vi "Convert API String Arguments to Data(variant).vi"(7 "Type":variant, 9 "error in (no error)":errorcluster, 10 "Strict Label Check?(T)":bool=TRUE, 11 "String":string) -> (1 "error":errorcluster, 3 "Data":variant)   [LabVIEW 2017, in "API String Arguments Support.lvlib"]
uses:
  API String Arguments Support.lvlib
  <vilib>/Utility/Data Type/Type Definitions/Data Type.ctl
  <vilib>/Utility/Data Type/Type Definitions/Tag Type.ctl
  <vilib>/Utility/Data Type/Type Definitions/Refnum Type.ctl
  <userlib>/_NEVSTOP/Communicable State Machine(CSM)/AdvanceAPI/CSM - Keywords.vi
  <vilib>/Utility/Data Type/NI_Data Type.lvlib
  <userlib>/_NEVSTOP/Communicable State Machine(CSM)/Communicable State Machine.lvlib
  <userlib>/_NEVSTOP/Communicable State Machine(CSM)/_Shared/CSM Shared.lvlib
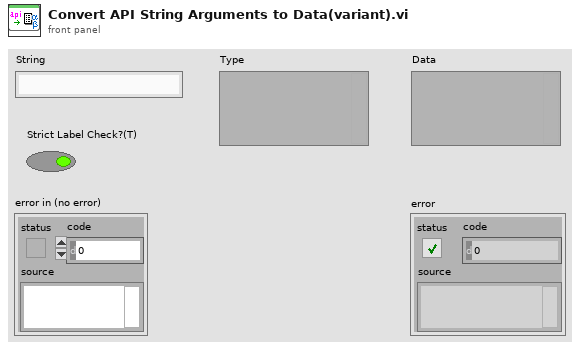
[diagram p1: front panel]
types:
  T1 = enum16{"0x2829 - ()", "0x5B5D - []", "0x7B7D - {}"}
  T2 = typedef "NI_Data Type.lvlib/Data Type.ctl" = enum8{"Invalid Type", "Void", "I8", "I16", "I32", "I64", "U8", "U16", "U32", "U64", "Single Float", "Double Float", "Extended Float", "Single Complex", "Double Complex", "Extended Complex", "Enum U8", "Enum U16", "Enum U32", "Enum U64", "Single Float With Unit", "Double Float With Unit", "Extended Float With Unit", "Single Complex with Unit", "Double Complex with Unit", "Extended Complex with Unit", "Boolean", "String", "Path", "Picture", "Tag", "Array", "Cluster", "Variant", "LV Variant", "Waveform", "Timestamp", "Digital Waveform", "Digital Data", "ExpressData", "Refnum", "External Data", "VI", "Poly VI", "LabVIEW Class Instance", "Fixed Point"}
  T3 = typedef "NI_Data Type.lvlib/Tag Type.ctl" = enum16{"kNoTagType", "\tkDSCTagType", "\tkOldDAQTagType", "\tkIVITagType", "\tkVISATagType", "\tkGenClassTagType", "\tkUnusedTagType1", "\tkFPTagType", "\tkMotionTagType", "\tkDAQmxTaskTagType", "\tkDAQmxChannelTagType", "\tkDAQmxScaleTagType", "\tkDAQmxDeviceTagType", "\tkDAQmxTerminalTagType", "\tkDAQmxPhysChanTagType", "\tkDAQmxTriggerTagType", "\tkDAQmxSwitchTagType", "\tkDAQmxSignalTagType", "\tkUnusedTagType2", "\tkCANTaskTagType", "\tkCANInterfaceTagType", "\tkCANChannelTagType", "\tkNumTagTypes"}
  T4 = typedef "NI_Data Type.lvlib/Refnum Type.ctl" = enum16{"NotARefnum", "UnknownRefnum", "Generic", "Datalog", "ByteStream", "Device", "Occurence", "TCPNetConnection", "Auto", "Menu", "Imaq", "Hardware", "DataSocket", "Visa", "IVI", "UDPNetConnection", "Notifier", "Queue", "Irda", "EventReg", "DotNet", "UserEvent", "Callback", "UNUSED_EMPTY_POSITION", "BlueToothNetConnection", "LVObjApp", "LVObjVI", "LVObjUnknown", "GenericClass", "UserDefinedRefnumTag", "DataValue", "RT FIFO", "TDMS File"}
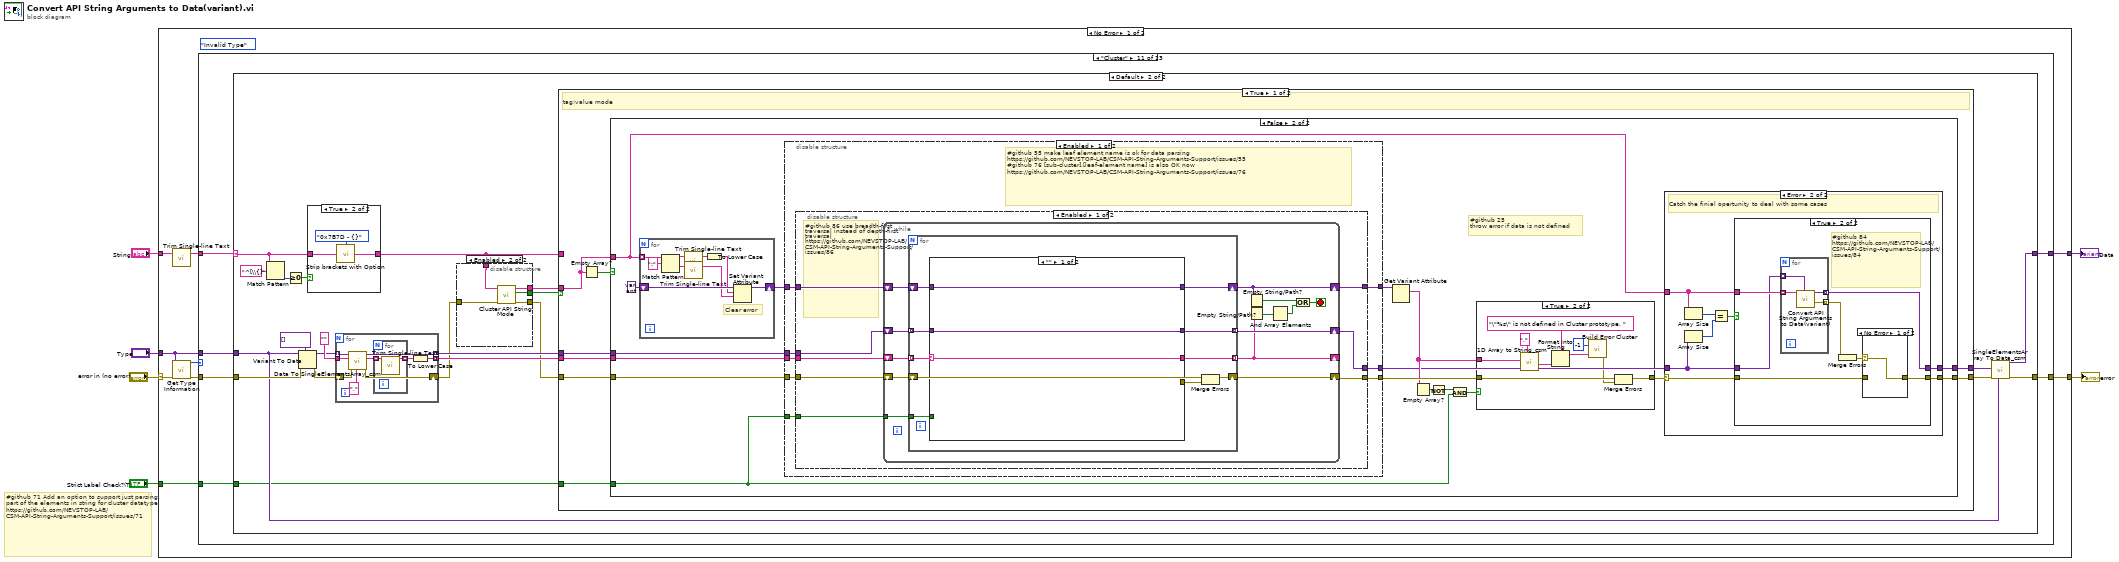
[diagram p0: block diagram]
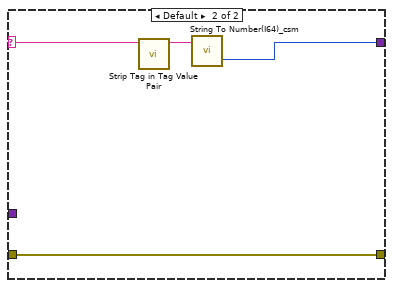
[diagram p3: hidden frame]
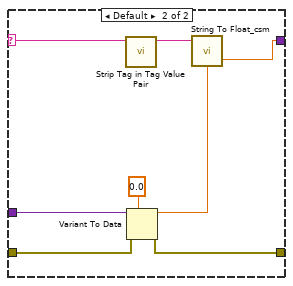
[diagram p5: hidden frame]
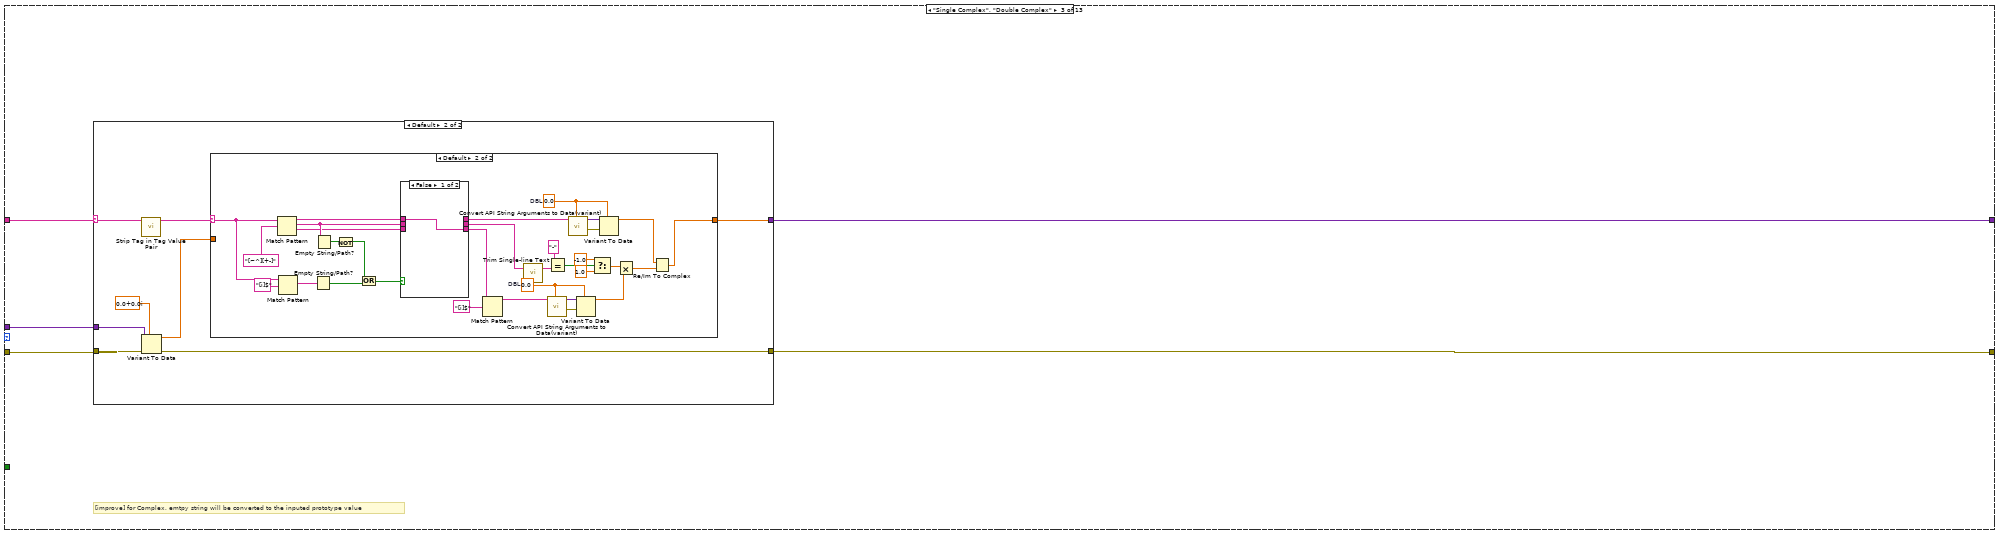
[diagram p6: hidden frame]
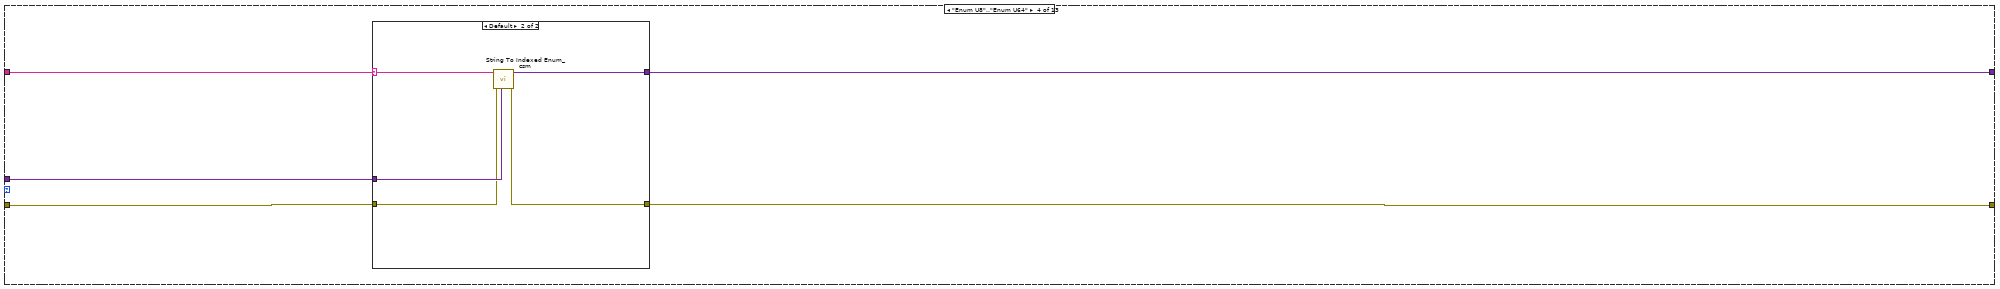
[diagram p10: hidden frame]
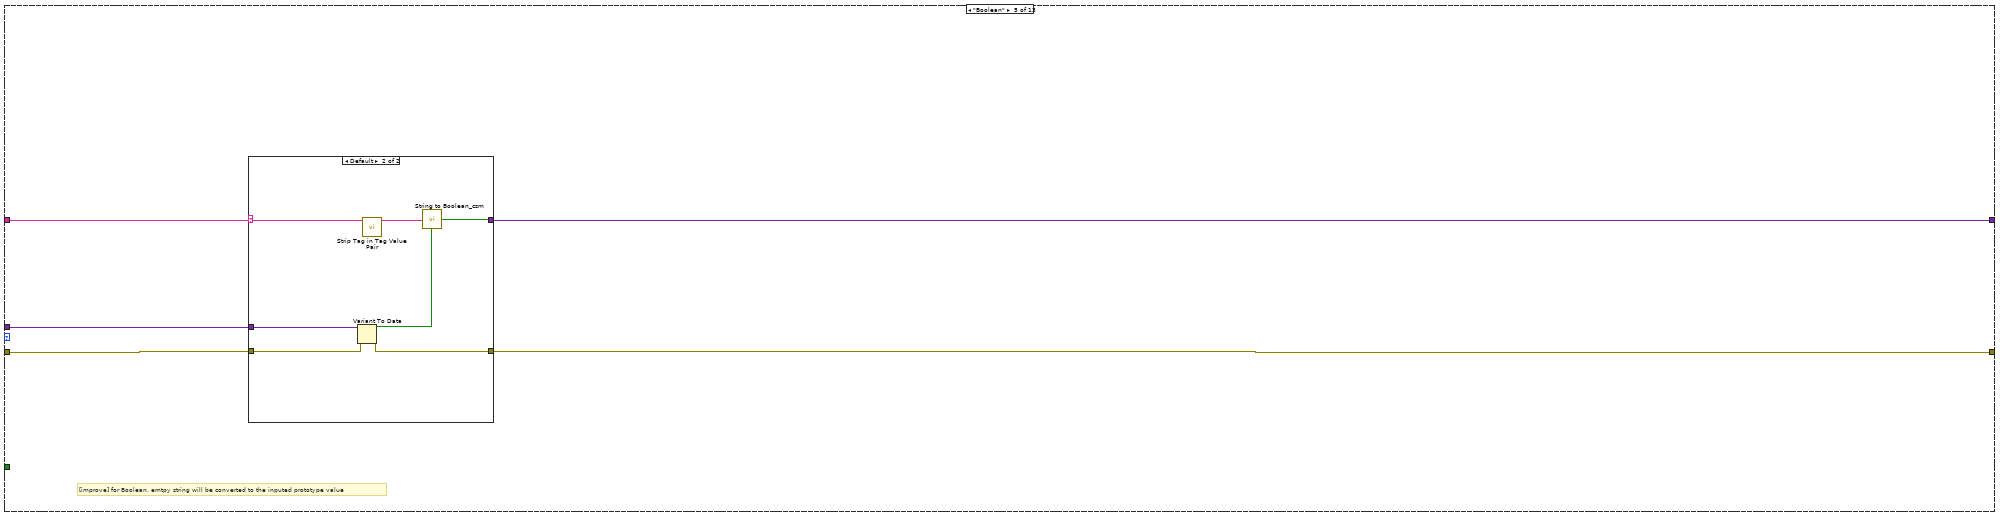
[diagram p12: hidden frame]
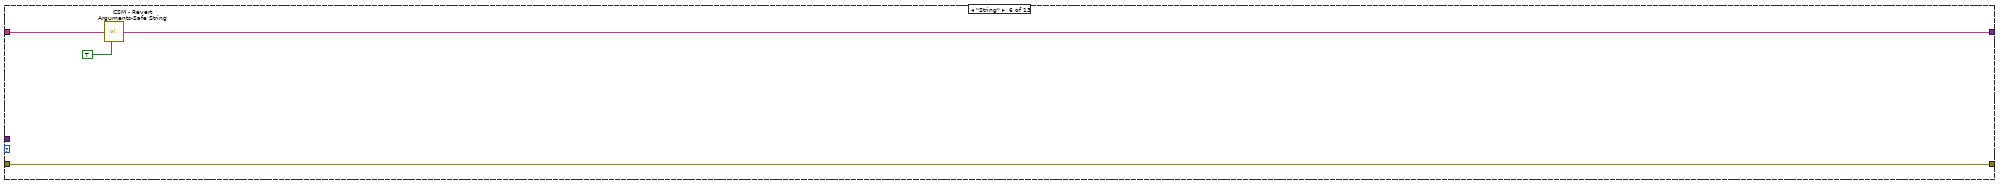
[diagram p14: hidden frame]
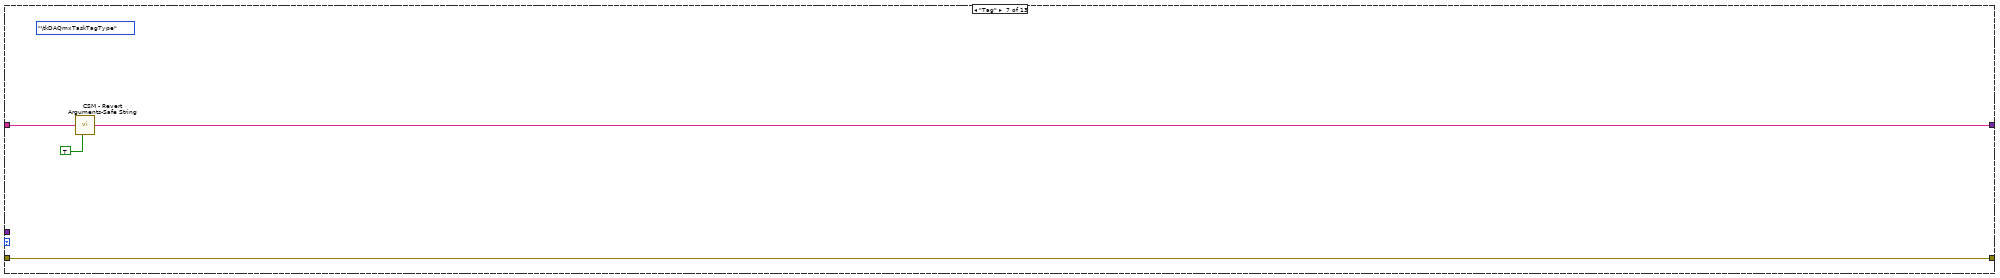
[diagram p15: hidden frame]
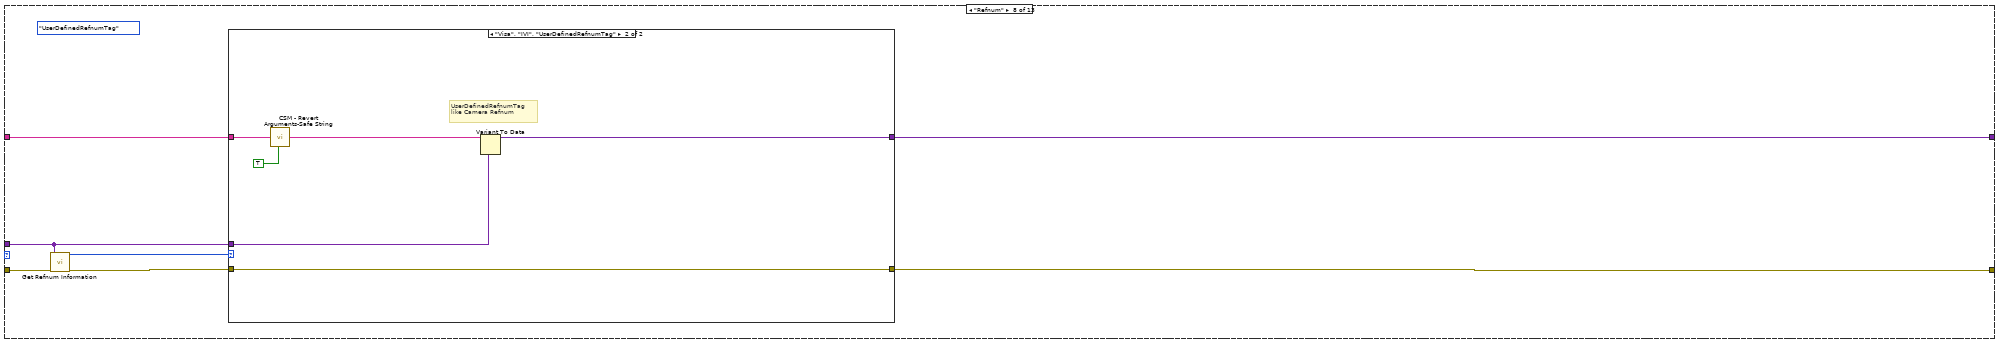
[diagram p16: hidden frame]
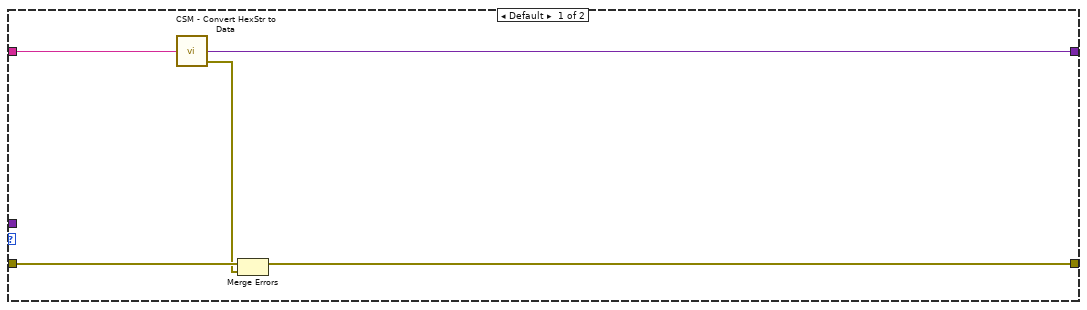
[diagram p17: hidden frame]
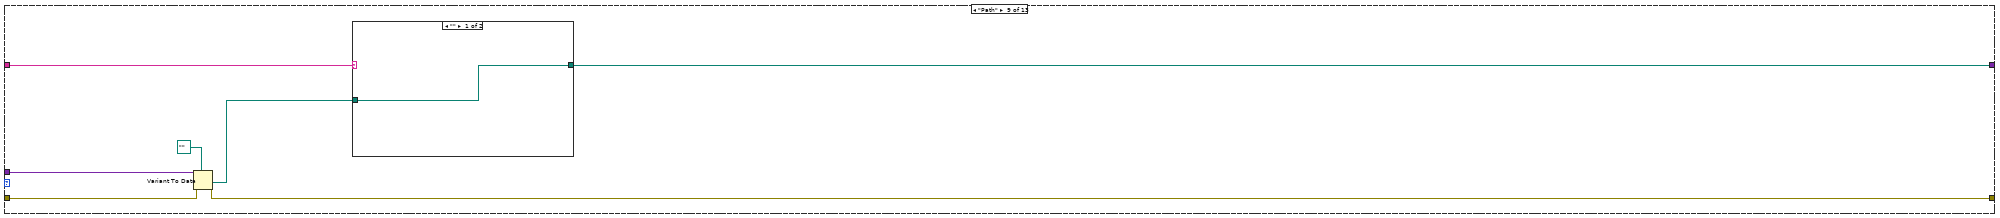
[diagram p18: hidden frame]
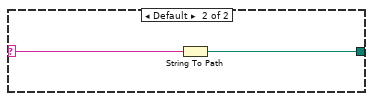
[diagram p19: hidden frame]
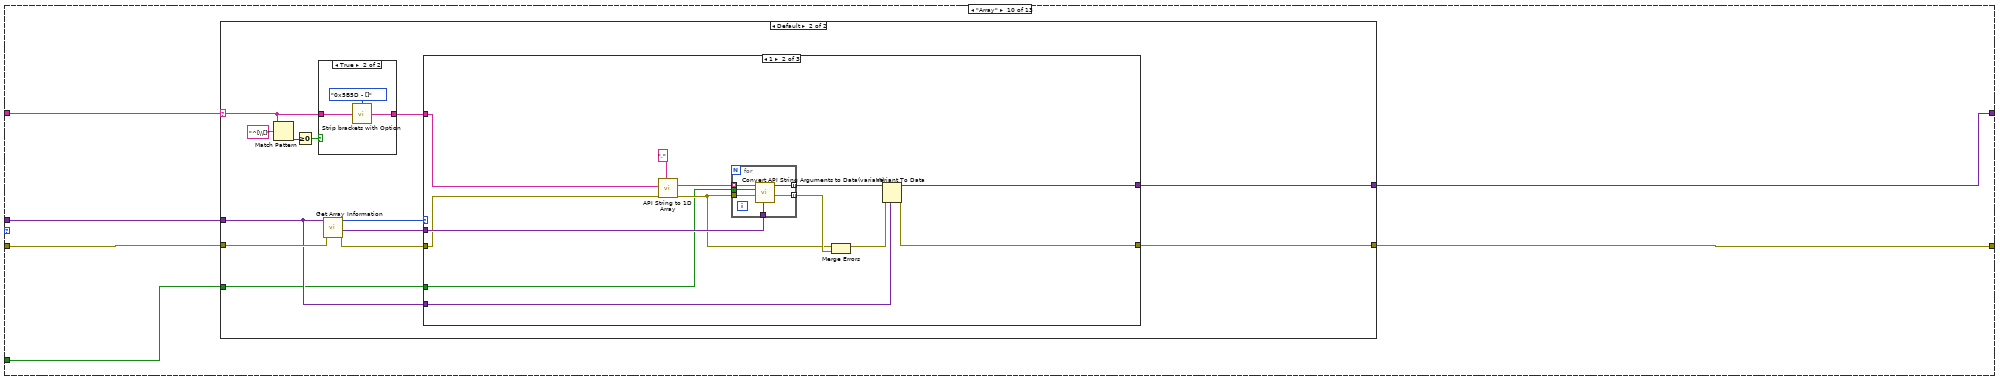
[diagram p20: hidden frame]
diagram:
  # "#github 71 Add an option to support just parsing part of the elements in string for cluster datatype\nhttps://github.com/NEVSTOP-LAB/CSM-API-String-Arguments-Support/issues/71"
  n1 = case shown="No Error" "error in (no error)" {
    selector: "error in (no error)" -> [w10 w622]
    tunnel: [w13 w622] -> w6
    tunnel: [w12 w621] -> w5
    tunnel: "Type" -> [w11 w621]
    tunnel: "String" -> [w9 _]
    tunnel: "Strict Label Check?(T)" -> [w7 _]
    frame No Error {
      (unwired) Data_Type."Invalid Type" ("type")
      n2 = call <userlib>:"Trim Single-line Text.vi"("single-line text"=w9) -> ("trimed text"=w8:string)  [unwired: 2 in]
      n3 = call <vilib>:"Get Type Information.vi"("error in (no error)"=w10, "Variant"=w11) -> ("error out"=w14:errorcluster, "Type"=w15:T2)  [unwired: 5 in, 3 out]
      n4 = case shown="\"Cluster\"" w15 {
        tunnel: w14 -> [w18 w31 w46 w96 w107 w123 w127 w134 w152 w161 w243 w573 w613]
        tunnel: [w17 w28 w44 w95 w106 w123 w127 w132 w149 w159 w246 w571 w610] -> w13
        tunnel: [w19 w29 w45 w94 w109 w121 w125 w129 w150 w160 w245 w572 w611] -> w12
        tunnel: w11 -> [w16 w27 w43 w97 w108 _ _ w131 w148 w158 w244 _ w609]
        tunnel: w8 -> [w20 w30 w42 w98 w110 w122 w126 w130 w151 w157 w242 w570 w612]
        tunnel: w7 -> [_ _ _ _ _ _ _ _ _ w156 w241 _ _]
        frame "I8".."U64" {
          # "For Integer, empty string will be converted to the input prototype value"
          n5 = case shown="\"\"" w20 {
            selector: w20 -> [_ w26]
            tunnel: [w22 w25] -> w19
            tunnel: w18 -> [w21 w24]
            tunnel: [w21 w24] -> w17
            tunnel: w16 -> [w22 _]
            frame "" {
            }
            frame Default {
              n6 = call "Strip Tag in Tag Value Pair.vi"("Tag:Value"=w26) -> ("Value"=w23:string)  [unwired: 10 in]
              n7 = call "String To Number(I64)_csm.vi"("String"=w23) -> ("Numeric"=w25:u64)  [unwired: 4 in]
            }
          }
        }
        frame "Single Float", "Double Float" {
          # "[improve] for SGL/DBL, emtpy string will be converted to the inputed prototype value"
          n8 = case shown="\"\"" w30 {
            selector: w30 -> [_ w40]
            tunnel: w31 -> [w33 w41]
            tunnel: [w32 w39] -> w29
            tunnel: [w33 w38] -> w28
            tunnel: w27 -> [w32 w37]
            frame "" {
            }
            frame Default {
              n9 = call "Strip Tag in Tag Value Pair.vi"("Tag:Value"=w40) -> ("Value"=w34:string)  [unwired: 10 in]
              n10 = Variant To Data(error in=w41, type=0.0 ("Default(0)"), Variant=w37) -> (data=w35:dbl, error out=w38:errorcluster)
              n11 = call "String To Float_csm.vi"("Default (0)"=w35, "String"=w34) -> ("Float"=w39:dbl)  [unwired: 2 in, 1 out]
            }
          }
        }
        frame "Single Complex", "Double Complex" {
          # "[improve] for Complex, emtpy string will be converted to the inputed prototype value"
          n12 = case shown="Default" w42 {
            selector: w42 -> [_ w50]
            tunnel: w46 -> [w48 w56]
            tunnel: [w47 w55] -> w45
            tunnel: [w48 w54] -> w44
            tunnel: w43 -> [w47 w53]
            frame "" {
            }
            frame Default {
              n13 = call "Strip Tag in Tag Value Pair.vi"("Tag:Value"=w50) -> ("Value"=w49:string)  [unwired: 10 in]
              n14 = Variant To Data(error in=w56, type=cdb 0.0+0.0i ("x + iy"), Variant=w53) -> (data=w51:cdb, error out=w54:errorcluster)
              n15 = case shown="Default" w49 {
                selector: w49 -> [_ w71]
                tunnel: [w57 w73] -> w55
                tunnel: w51 -> [w57 _]
                frame "" {
                }
                frame Default {
                  w82 = 0.0  # DBL
                  w85 = 0.0  # DBL
                  n16 = Match Pattern(string=w71, regular expression="[~^][+-]") -> (before substring=w66:string, match substring=w62:string, after substring=w61:string)  [unwired: 1 in, 1 out]
                  n17 = Match Pattern(string=w71, regular expression="[i]$") -> (match substring=w69:string)  [unwired: 1 in, 3 out]
                  n18 = Empty String/Path?(string/path=w69) -> (empty?=w63:bool)
                  n19 = Empty String/Path?(string/path=w62) -> (empty?=w68:bool)
                  n20 = Not(x=w68) -> (.not. x?=w64:bool)
                  n21 = Or(x=w64, y=w63) -> (x .or. y?=w67:bool)
                  n22 = case shown="False" w67 {
                    tunnel: w66 -> [w90 w93]
                    tunnel: [_ w93] -> w65
                    tunnel: w62 -> [_ w92]
                    tunnel: [_ w92] -> w58
                    tunnel: w61 -> [_ w91]
                    tunnel: [w90 w91] -> w60
                    frame False {
                    }
                    frame True {
                    }
                  }
                  n23 = Match Pattern(string=w60, regular expression="[i]$") -> (before substring=w72:string)  [unwired: 1 in, 3 out]
                  n24 = call <userlib>:"Trim Single-line Text.vi"("single-line text"=w58) -> ("trimed text"=w59:string)  [unwired: 2 in]
                  n25 = call "Convert API String Arguments to Data(variant).vi"("Type"=w82, "String"=w72) -> ("error"=w84:errorcluster, "Data"=w83:variant)  [unwired: 8 in]
                  n26 = Equal?(x="-", y=w59) -> (x = y?=w79:bool)
                  n27 = call "Convert API String Arguments to Data(variant).vi"("Type"=w85, "String"=w65) -> ("error"=w87:errorcluster, "Data"=w86:variant)  [unwired: 8 in]
                  n28 = Variant To Data(error in=w84, type=w82, Variant=w83) -> (data=w81:dbl)  [unwired: 1 out]
                  n29 = Select(t=-1.0, s=w79, f=1.0 ("t")) -> (s? t:f=w78:dbl)
                  n30 = Variant To Data(error in=w87, type=w85, Variant=w86) -> (data=w74:dbl)  [unwired: 1 out]
                  n31 = Multiply(x=w78, y=w81) -> (x*y=w75:dbl)
                  n32 = Re/Im To Complex(1:w75, 2:w74) -> (0:w73:cdb)
                }
              }
            }
          }
        }
        frame "Enum U8".."Enum U64" {
          n33 = case shown="Default" w98 {
            selector: w98 -> [_ w105]
            tunnel: w97 -> [w100 w104]
            tunnel: w96 -> [w99 w103]
            tunnel: [w99 w102] -> w95
            tunnel: [w100 w101] -> w94
            frame "" {
            }
            frame Default {
              n34 = call "String To Indexed Enum_csm.vi"("Variant"=w104, "error in (no error)"=w103, "String"=w105) -> ("error out"=w102:errorcluster, "Enum"=w101:variant)  [unwired: 7 in]
            }
          }
        }
        frame "Boolean" {
          # "[improve] for Boolean, emtpy string will be converted to the inputed prototype value"
          n35 = case shown="Default" w110 {
            selector: w110 -> [_ w119]
            tunnel: [w112 w118] -> w109
            tunnel: w108 -> [w112 w117]
            tunnel: w107 -> [w111 w115]
            tunnel: [w111 w114] -> w106
            frame "" {
            }
            frame Default {
              n36 = Variant To Data(error in=w115, Variant=w117) -> (data=w116:bool, error out=w114:errorcluster)  [unwired: 1 in]
              n37 = call "Strip Tag in Tag Value Pair.vi"("Tag:Value"=w119) -> ("Value"=w113:string)  [unwired: 10 in]
              n38 = call "String to Boolean_csm.vi"("Default (F)"=w116, "String"=w113) -> ("Boolean"=w118:bool)  [unwired: 2 in]
            }
          }
        }
        frame "String" {
          n39 = call <userlib>:"CSM - Revert Arguments-Safe String.vi"("Safe Argument String"=w122, "Force Convert (F)"=TRUE) -> ("Origin Argument String"=w121:string)  [unwired: 7 in]
        }
        frame "Tag" {
          (unwired) Tag_Type."\tkDAQmxTaskTagType" ("Tag Type")
          n40 = call <userlib>:"CSM - Revert Arguments-Safe String.vi"("Safe Argument String"=w126, "Force Convert (F)"=TRUE) -> ("Origin Argument String"=w125:string)  [unwired: 7 in]
        }
        frame "Refnum" {
          (unwired) Refnum_Type."UserDefinedRefnumTag" ("Reference Type")
          n41 = call <vilib>:"Get Refnum Information.vi"("error in (no error)"=w134, "Variant"=w131) -> ("error out"=w133:errorcluster, "Reference Type"=w128:T4)  [unwired: 6 in, 2 out]
          n42 = case shown="\"Visa\", \"IVI\", \"UserDefinedRefnumTag\"" w128 {
            tunnel: w133 -> [w139 w145]
            tunnel: [w137 w143] -> w129
            tunnel: [w136 w145] -> w132
            tunnel: w131 -> [_ w144]
            tunnel: w130 -> [w138 w142]
            frame Default {
              n43 = call <userlib>:"CSM - Convert HexStr to Data.vi"("HEX String"=w138) -> ("Variant"=w137:variant, "error out"=w135:errorcluster)  [unwired: 7 in]
              n44 = Merge Errors(w139, w135) -> (w136:errorcluster)
            }
            frame "Visa", "IVI", "UserDefinedRefnumTag" {
              # "UserDefinedRefnumTag\nlike Camera Refnum"
              n45 = call <userlib>:"CSM - Revert Arguments-Safe String.vi"("Safe Argument String"=w142, "Force Convert (F)"=TRUE) -> ("Origin Argument String"=w141:string)  [unwired: 7 in]
              n46 = Variant To Data(type=w144, Variant=w141) -> (data=w143:variant)  [unwired: 1 in, 1 out]
            }
          }
        }
        frame "Path" {
          n47 = Variant To Data(error in=w152, type=path "", Variant=w148) -> (data=w146:path, error out=w149:errorcluster)
          n48 = case shown="\"\"" w151 {
            selector: w151 -> [_ w155]
            tunnel: [w153 w154] -> w150
            tunnel: w146 -> [w153 _]
            frame "" {
            }
            frame Default {
              n49 = String To Path(string=w155) -> (path=w154:path)
            }
          }
        }
        frame "Array" {
          n50 = case shown="Default" w157 {
            selector: w157 -> [_ w166]
            tunnel: w161 -> [w163 w176]
            tunnel: [w162 w175] -> w160
            tunnel: [w163 w174] -> w159
            tunnel: w158 -> [w162 w170]
            tunnel: w156 -> [_ w164]
            frame "" {
            }
            frame Default {
              n51 = Match Pattern(string=w166, regular expression="^[\\[]") -> (offset past match=w169:i32)  [unwired: 1 in, 3 out]
              n52 = Greater Or Equal To 0?(x=w169) -> (x >= 0?=w168:bool)
              n53 = case shown="True" w168 {
                tunnel: [w237 w238] -> w165
                tunnel: w166 -> [w237 w240]
                frame False {
                }
                frame True {
                  n54 = call "Strip brackets with Option.vi"("TYPE"=T1."0x5B5D - []", "trimmed string in"=w240) -> ("trimmed string out"=w238:string)  [unwired: 2 in]
                }
              }
              n55 = call <vilib>:"Get Array Information.vi"("error in (no error)"=w176, "Variant"=w170) -> ("error out"=w173:errorcluster, "Array Element Data Type"=w172:variant, "Number of Dimensions"=w171:i32)  [unwired: 6 in, 1 out]
              n56 = case shown="1" w171 {
                tunnel: w165 -> [_ w180 w202]
                tunnel: [w178 w190 w210] -> w175
                tunnel: [errorcluster {"status"=TRUE, "code"=-1, "source"="DataType is not supported."} ("error out") w188 w208] -> w174
                tunnel: w173 -> [_ w184 w207]
                tunnel: w172 -> [_ w187 w203]
                tunnel: w170 -> [w178 w185 w206]
                tunnel: w164 -> [_ w179 w198]
                frame Default {
                }
                frame 1 {
                  n57 = call "API String to 1D Array.vi"("delimiter"="," ("delimiter (Tab)"), "error in (no error)"=w184, "trimmed string in"=w180) -> ("error out"=w183:errorcluster, "Array of Strings"=w181:string[])  [unwired: 7 in]
                  n58 = for {
                    tunnel: w181 -> [w194] mode=indexing
                    tunnel: [w196] -> w191 mode=indexing
                    tunnel: [w195] -> w186 mode=indexing
                    tunnel: w187 -> [w197]
                    tunnel: w183 -> [w193]
                    tunnel: w179 -> [w192]
                    n59 = call "Convert API String Arguments to Data(variant).vi"("Type"=w197, "error in (no error)"=w193, "Strict Label Check?(T)"=w192, "String"=w194) -> ("error"=w196:errorcluster, "Data"=w195:variant)  [unwired: 6 in]
                  }
                  n60 = Merge Errors(w183, w191) -> (w189:errorcluster)
                  n61 = Variant To Data(error in=w189, type=w185, Variant=w186) -> (data=w190:variant, error out=w188:errorcluster)
                }
                frame 2 {
                  n62 = call "API String to 1D Array.vi"("delimiter"=";" ("delimiter (Tab)"), "error in (no error)"=w207, "trimmed string in"=w202) -> ("error out"=w199:errorcluster, "Array of Strings"=w200:string[])  [unwired: 7 in]
                  n63 = for {
                    tunnel: [w220] -> w205 mode=indexing
                    tunnel: w203 -> [w219]
                    shift-right: [w221] -> w209
                    shift-left: w199 -> [w213]
                    tunnel: w200 -> [w215] mode=indexing
                    tunnel: w198 -> [w211]
                    n64 = call <userlib>:"Trim Single-line Text.vi"("single-line text"=w215) -> ("trimed text"=w214:string)  [unwired: 2 in]
                    n65 = call "API String to 1D Array.vi"("delimiter"="," ("delimiter (Tab)"), "error in (no error)"=w213, "trimmed string in"=w214) -> ("error out"=w212:errorcluster, "Array of Strings"=w217:string[])  [unwired: 7 in]
                    n66 = for {
                      tunnel: w217 -> [w225] mode=indexing
                      tunnel: [w227] -> w216 mode=indexing
                      tunnel: [w226] -> w220 mode=indexing
                      tunnel: w219 -> [w228]
                      tunnel: w212 -> [w223]
                      tunnel: w211 -> [w222]
                      n67 = call <userlib>:"Trim Single-line Text.vi"("single-line text"=w225) -> ("trimed text"=w224:string)  [unwired: 2 in]
                      n68 = call "Convert API String Arguments to Data(variant).vi"("Type"=w228, "error in (no error)"=w223, "Strict Label Check?(T)"=w222, "String"=w224) -> ("error"=w227:errorcluster, "Data"=w226:variant)  [unwired: 6 in]
                    }
                    n69 = Merge Errors(w212, w216) -> (w221:errorcluster)
                  }
                  n70 = for {
                    tunnel: w205 -> [w231] mode=indexing
                    tunnel: [w230] -> w204 mode=indexing
                    tunnel: w203 -> [w229]
                    n71 = for {
                      tunnel: w231 -> [w233] mode=indexing
                      tunnel: [w232] -> w230 mode=indexing
                      tunnel: w229 -> [w234]
                      n72 = Not Equal?(x=w233, y=variant ("Data")) -> (x != y?=w235:bool)
                      n73 = Select(t=w233, s=w235, f=w234) -> (s? t:f=w232:variant)
                    }
                  }
                  n74 = Variant To Data(error in=w209, type=w206, Variant=w204) -> (data=w210:variant, error out=w208:errorcluster)
                }
              }
            }
          }
        }
        frame "Cluster" {
          n75 = case shown="Default" w242 {
            selector: w242 -> [_ w260]
            tunnel: [w247 w269] -> w246
            tunnel: [w248 w267] -> w245
            tunnel: w244 -> [w248 w259]
            tunnel: w243 -> [w247 w262]
            tunnel: w241 -> [_ w253]
            frame "" {
            }
            frame Default {
              n76 = Match Pattern(string=w260, regular expression="^[\\{]") -> (offset past match=w265:i32)  [unwired: 1 in, 3 out]
              n77 = Greater Or Equal To 0?(x=w265) -> (x >= 0?=w264:bool)
              n78 = Variant To Data(error in=w262, type=variant[] [] ("Array"), Variant=w259) -> (data=w257:variant[], error out=w255:errorcluster)
              n79 = case shown="True" w264 {
                tunnel: [w566 w567] -> w261
                tunnel: w260 -> [w566 w569]
                frame False {
                }
                frame True {
                  n80 = call "Strip brackets with Option.vi"("TYPE"=T1."0x7B7D - {}", "trimmed string in"=w569) -> ("trimmed string out"=w567:string)  [unwired: 2 in]
                }
              }
              n81 = for {
                tunnel: [w561] -> w256 mode=concatenating
                tunnel: [w555] -> w254 mode=concatenating
                tunnel: "" ("parentUrl") -> [w558]
                tunnel: w257 -> [w557] mode=indexing
                shift-right: [w560] -> w250
                shift-left: w255 -> [w563]
                n82 = call "Data To SingleElementsArray_csm.vi"("Seperator(/)"=".", "error in (no error)"=w563, "parentUrl"=w558, "Cluster"=w557) -> ("error out"=w560:errorcluster, "Full NameList"=w559:string[], "DataElementArray"=w561:variant[])  [unwired: 5 in]
                n83 = for {
                  tunnel: w559 -> [w565] mode=indexing
                  tunnel: [w564] -> w556 mode=indexing
                  n84 = call <userlib>:"Trim Single-line Text.vi"("single-line text"=w565) -> ("trimed text"=w564:string)  [unwired: 2 in]
                }
                n85 = To Lower Case(string=w556) -> (all lower case string=w555:string[])
              }
              n86 = disable-structure shown="Enabled" {
                disable-tunnel: w261 -> [w548 w554]
                disable-tunnel: [w546 w553] -> w252
                disable-tunnel: [_ w552] -> w251
                disable-tunnel: w250 -> [w545 w551]
                disable-tunnel: [w545 w550] -> w249
                frame Disabled {
                  # "#github 23\n判断是否只有Label:Value Pair"
                  n87 = Match Pattern(string=w548, regular expression=":") -> (offset past match=w547:i32)  [unwired: 1 in, 3 out]
                  n88 = Greater Or Equal To 0?(x=w547) -> (x >= 0?=w546:bool)
                }
                frame Enabled {
                  n89 = call "Cluster API String Mode.vi"("error in (no error)"=w551, "cluster api string"=w554) -> ("error out"=w550:errorcluster, "TagValue Mode"=w553:bool, "Array of Strings"=w552:string[])  [unwired: 7 in]
                }
              }
              n90 = case shown="True" w252 {
                tunnel: [w278 w509] -> w270
                tunnel: [w277 w510] -> w268
                tunnel: w249 -> [w272 w504]
                tunnel: w261 -> [_ w506]
                tunnel: w256 -> [w276 w503]
                tunnel: w254 -> [w275 _]
                tunnel: w253 -> [w274 w502]
                tunnel: w251 -> [w271 _]
                frame True {
                  # "tag:value mode"
                  n91 = Empty Array?(array=w271) -> (empty?=w273:bool)
                  n92 = case shown="False" w273 {
                    tunnel: [w279 w282] -> w278
                    tunnel: [w280 w285] -> w277
                    tunnel: w276 -> [w279 w295]
                    tunnel: w275 -> [_ w294]
                    tunnel: w272 -> [w280 w293]
                    tunnel: w274 -> [_ w288]
                    tunnel: w271 -> [_ w281]
                    frame True {
                    }
                    frame False {
                      # "#github 25\nthrow error if data is not defined"
                      n93 = for {
                        tunnel: w281 -> [w499] mode=indexing
                        shift-right: [w500] -> w296
                        shift-left: variant -> [w501]
                        # "Clear error"
                        n94 = Match Pattern(string=w499, regular expression=":") -> (before substring=w496:string, after substring=w497:string)  [unwired: 1 in, 2 out]
                        n95 = call <userlib>:"Trim Single-line Text.vi"("single-line text"=w496) -> ("trimed text"=w494:string)  [unwired: 2 in]
                        n96 = call <userlib>:"Trim Single-line Text.vi"("single-line text"=w497) -> ("trimed text"=w495:string)  [unwired: 2 in]
                        n97 = To Lower Case(string=w494) -> (all lower case string=w493:string)
                        n98 = Set Variant Attribute(Variant=w501, name=w493, value=w495) -> (Variant out=w500:variant)  [unwired: 1 in, 2 out]
                      }
                      n99 = disable-structure shown="Enabled" {
                        disable-tunnel: w296 -> [w330 w444]
                        disable-tunnel: [w329 w443] -> w283
                        disable-tunnel: w295 -> [w328 w442]
                        disable-tunnel: w294 -> [w327 w441]
                        disable-tunnel: w293 -> [w326 w440]
                        disable-tunnel: [w325 w439] -> w292
                        disable-tunnel: w288 -> [w324 w438]
                        disable-tunnel: [w323 w436] -> w287
                        frame Enabled {
                          # "#github 55 make leaf element name is ok for data parsing \nhttps://github.com/NEVSTOP-LAB/CSM-API-String-Arguments-Support/issues/55 \n#github 76 [sub-cluster].[leaf-element name] is also OK now\nhttps://github.com/NEVSTOP-LAB/CSM-API-String-Arguments-Support/issues/76"
                          n100 = disable-structure shown="Enabled" {
                            disable-tunnel: w330 -> [w338 w398]
                            disable-tunnel: [w332 w397] -> w329
                            disable-tunnel: w328 -> [w337 w396]
                            disable-tunnel: w327 -> [w331 w395]
                            disable-tunnel: w326 -> [w336 w394]
                            disable-tunnel: [w335 w393] -> w325
                            disable-tunnel: w324 -> [w334 w392]
                            disable-tunnel: [w333 w390] -> w323
                            frame Enabled {
                              # "#github 86 use breadth-first traversal instead of depth-first traversal \nhttps://github.com/NEVSTOP-LAB/CSM-API-String-Arguments-Support/issues/86"
                              n101 = while {
                                shift-right: [w344] -> w335
                                shift-left: w338 -> [w351]
                                tunnel: w334 -> [w350]
                                shift-right: [w348] -> w332
                                shift-left: w337 -> [w349]
                                shift-right: [w343] -> _
                                shift-left: w331 -> [w347]
                                shift-right: [w346] -> w333
                                shift-left: w336 -> [w345]
                                stop <- w342 stop-if-true
                                n102 = for {
                                tunnel: w350 -> [w358]
                                shift-right: [w359] -> w344
                                shift-left: w351 -> [w361]
                                shift-right: [w357] -> w346
                                shift-left: w345 -> [w356]
                                tunnel: w349 -> [w354] mode=indexing
                                tunnel: [w352] -> w348 mode=indexing
                                tunnel: w347 -> [w355] mode=indexing
                                tunnel: [w353] -> w343 mode=indexing
                                n103 = case shown="\"\"" w355 {
                                selector: w355 -> [w362 w366]
                                tunnel: w361 -> [w364 w376]
                                tunnel: [_ w375] -> w360
                                tunnel: [w364 w373] -> w359
                                tunnel: w358 -> [_ w372]
                                tunnel: w354 -> [w363 w371]
                                tunnel: [w363 w370] -> w352
                                tunnel: [w362 w365] -> w353
                                frame "" {
                                }
                                frame Default {
                                n104 = Get Variant Attribute(Variant=w376, name=w366, default value (empty Variant)="" ("regular expression")) -> (duplicate Variant=w368:variant, found=w367:bool, value=w374:string)  [unwired: 1 in, 1 out]
                                n105 = case shown="False" w367 {
                                tunnel: [_ w389] -> w375
                                tunnel: w374 -> [_ w388]
                                tunnel: [w380 w387] -> w373
                                tunnel: w372 -> [_ w386]
                                tunnel: w371 -> [w381 w385]
                                tunnel: [w381 w384] -> w370
                                tunnel: w366 -> [_ w383]
                                tunnel: w368 -> [w380 w382]
                                tunnel: w366 -> [w379 _]
                                tunnel: [w377 _] -> w365
                                frame False {
                                n106 = Match Pattern(string=w379, regular expression="[.]" ("delimiter (Tab)")) -> (after substring=w377:string)  [unwired: 1 in, 3 out]
                                }
                                frame True {
                                n107 = call "Convert API String Arguments to Data(variant).vi"("Type"=w385, "Strict Label Check?(T)"=w386, "String"=w388) -> ("error"=w389:errorcluster, "Data"=w384:variant)  [unwired: 7 in]
                                n108 = Delete Variant Attribute(6:w383, 7:w382) -> (3:w387:variant)  [unwired: 1 in, 2 out]
                                }
                                }
                                }
                                }
                                n109 = Merge Errors(w356, w360) -> (w357:errorcluster)
                                }
                                n110 = Empty String/Path?(string/path=w344) -> (empty?=w341:bool)
                                n111 = Empty String/Path?(string/path=w343) -> (empty?=w340:bool[])
                                n112 = And Array Elements(Boolean array=w340) -> (logical AND=w339:bool)
                                n113 = Or(x=w341, y=w339) -> (x .or. y?=w342:bool)
                              }
                            }
                            frame Disabled {
                              n114 = for {
                                tunnel: w396 -> [w408] mode=indexing
                                tunnel: w394 -> [w400]
                                tunnel: w395 -> [w405] mode=indexing
                                tunnel: [w407] -> w397 mode=indexing
                                tunnel: [w406] -> w391 mode=indexing
                                shift-right: [w402] -> w393
                                shift-left: w398 -> [w409]
                                tunnel: w392 -> [w401]
                                n115 = while {
                                tunnel: [w413] -> w403
                                shift-right: [w423] -> w402
                                shift-left: w409 -> [w420]
                                tunnel: [w424] -> w404
                                shift-right: [w418] -> _
                                shift-left: w405 -> [w417]
                                shift-right: [w410] -> w399
                                shift-left: w400 -> [w411]
                                stop <- w416 stop-if-true
                                n116 = Match Pattern(string=w417, regular expression="[.]" ("delimiter (Tab)")) -> (after substring=w418:string, offset past match=w415:i32)  [unwired: 1 in, 2 out]
                                n117 = Get Variant Attribute(Variant=w420, name=w417, default value (empty Variant)="" ("regular expression"), error in=w411) -> (duplicate Variant=w421:variant, found=w413:bool, value=w424:string, error out=w410:errorcluster)
                                n118 = Less Than 0?(x=w415) -> (x < 0?=w414:bool)
                                n119 = Or(x=w413, y=w410) -> (x .or. y?=w412:bool)
                                n120 = case shown="True" w413 {
                                tunnel: [w425 w428] -> w423
                                tunnel: w421 -> [w425 w427]
                                tunnel: w417 -> [_ w426]
                                frame False {
                                }
                                frame True {
                                n121 = Delete Variant Attribute(6:w426, 7:w427) -> (3:w428:variant)  [unwired: 1 in, 2 out]
                                }
                                }
                                n122 = Or(x=w412, y=w414) -> (x .or. y?=w416:bool)
                                }
                                n123 = case shown="True" w403 {
                                tunnel: w408 -> [w430 w435]
                                tunnel: w404 -> [_ w432]
                                tunnel: [w430 w434] -> w407
                                tunnel: [w429 w433] -> w406
                                tunnel: w399 -> [w429 _]
                                tunnel: w401 -> [_ w431]
                                frame False {
                                }
                                frame True {
                                n124 = call "Convert API String Arguments to Data(variant).vi"("Type"=w435, "Strict Label Check?(T)"=w431, "String"=w432) -> ("error"=w433:errorcluster, "Data"=w434:variant)  [unwired: 7 in]
                                }
                                }
                              }
                              n125 = Merge Errors(w391) -> (w390:errorcluster)
                            }
                          }
                        }
                        frame Disabled {
                          n126 = for {
                            tunnel: w442 -> [w456] mode=indexing
                            tunnel: w440 -> [w447]
                            tunnel: w441 -> [w452] mode=indexing
                            tunnel: [w455] -> w443 mode=indexing
                            tunnel: [w454] -> w437 mode=indexing
                            shift-right: [w446] -> w439
                            shift-left: w444 -> [w458]
                            tunnel: w438 -> [w445]
                            # "#github 55 make leaf element name is ok for data parsing \nhttps://github.com/NEVSTOP-LAB/CSM-API-String-Arguments-Support/issues/55"
                            n127 = Get Variant Attribute(Variant=w458, name=w452, default value (empty Variant)="" ("regular expression")) -> (duplicate Variant=w453:variant, found=w451:bool, value=w450:string)  [unwired: 1 in, 1 out]
                            n128 = case shown="False" w451 {
                              tunnel: w453 -> [w469 w473]
                              tunnel: w452 -> [w468 w471]
                              tunnel: w450 -> [_ w475]
                              tunnel: [w462 w475] -> w449
                              tunnel: [w463 TRUE] -> w448
                              tunnel: [w459 w472] -> w446
                              frame False {
                                n129 = call <userlib>:"String to 1D Array_csm.vi"("delimiter (Tab)"=".", "string"=w468) -> ("Array of Strings"=w465:string[])  [unwired: 9 in]
                                n130 = Array Size(array=w465) -> (size(s)=w466:i32)
                                n131 = Decrement(x=w466) -> (x-1=w464:i32)
                                n132 = Index Array(array=w465, index=w464) -> (element=w461:string)
                                n133 = Get Variant Attribute(Variant=w469, name=w461, default value (empty Variant)="" ("regular expression")) -> (duplicate Variant=w460:variant, found=w463:bool, value=w462:string)  [unwired: 1 in, 1 out]
                                n134 = Delete Variant Attribute(6:w461, 7:w460) -> (3:w459:variant)  [unwired: 1 in, 2 out]
                              }
                              frame True {
                                n135 = Delete Variant Attribute(6:w471, 7:w473) -> (3:w472:variant)  [unwired: 1 in, 2 out]
                              }
                            }
                            n136 = case shown="True" w448 {
                              tunnel: w456 -> [w477 w482]
                              tunnel: w449 -> [_ w479]
                              tunnel: [w477 w481] -> w455
                              tunnel: [w476 w480] -> w454
                              tunnel: w447 -> [w476 _]
                              tunnel: w445 -> [_ w478]
                              frame False {
                              }
                              frame True {
                                n137 = call "Convert API String Arguments to Data(variant).vi"("Type"=w482, "Strict Label Check?(T)"=w478, "String"=w479) -> ("error"=w480:errorcluster, "Data"=w481:variant)  [unwired: 7 in]
                              }
                            }
                          }
                          n138 = Merge Errors(w437) -> (w436:errorcluster)
                        }
                      }
                      n139 = Get Variant Attribute(Variant=w292) -> (names=w284:string[])  [unwired: 3 in, 3 out]
                      n140 = Empty Array?(array=w284) -> (empty?=w290:bool)
                      n141 = Not(x=w290) -> (.not. x?=w289:bool)
                      n142 = And(x=w289, y=w288) -> (x .and. y?=w291:bool)
                      n143 = case shown="True" w291 {
                        tunnel: w287 -> [w483 w492]
                        tunnel: [w483 w487] -> w286
                        tunnel: w284 -> [_ w485]
                        frame False {
                        }
                        frame True {
                          n144 = call <userlib>:"1D Array to String_csm.vi"("delimiter (Tab)"=",", "Array of Strings"=w485) -> ("delimited string"=w486:string)  [unwired: 9 in]
                          n145 = Format Into String(format string="\"%s\" is not defined in Cluster prototype. ", w486) -> (resulting string=w489:string)  [unwired: 2 in, 1 out]
                          n146 = call <userlib>:"Build Error Cluster.vi"("String to Prepend to Source (\"\")"=w489, "Code"=-1 ("code")) -> ("error out"=w491:errorcluster)
                          n147 = Merge Errors(w492, w491) -> (w487:errorcluster)
                        }
                      }
                      n148 = case shown="Error" w286 {
                        selector: w286 -> [w299 w303]
                        tunnel: [w299 w302] -> w285
                        tunnel: w281 -> [_ w306]
                        tunnel: w283 -> [w298 w304]
                        tunnel: [w298 w305] -> w282
                        frame No Error {
                        }
                        frame Error {
                          # "Catch the finial opertunity to deal with some cases"
                          n149 = Array Size(array=w306) -> (size(s)=w307:i32)
                          n150 = Array Size(array=w304) -> (size(s)=w301:i32)
                          n151 = Equal?(x=w307, y=w301) -> (x = y?=w300:bool)
                          n152 = case shown="True" w300 {
                            tunnel: w306 -> [_ w316]
                            tunnel: [w309 w314] -> w305
                            tunnel: w304 -> [w309 w315]
                            tunnel: w303 -> [w308 w310]
                            tunnel: [w308 w311] -> w302
                            frame False {
                            }
                            frame True {
                              # "#github 84 \nhttps://github.com/NEVSTOP-LAB/CSM-API-String-Arguments-Support/issues/84"
                              n153 = for {
                                tunnel: w316 -> [w322] mode=indexing
                                tunnel: w315 -> [w321] mode=indexing
                                tunnel: [w320] -> w314 mode=indexing
                                tunnel: [w319] -> w313 mode=indexing
                                n154 = call "Convert API String Arguments to Data(variant).vi"("Type"=w321, "String"=w322) -> ("error"=w319:errorcluster, "Data"=w320:variant)  [unwired: 8 in]
                              }
                              n155 = Merge Errors(w313) -> (w312:errorcluster)
                              n156 = case shown="No Error" w312 {
                                selector: w312 -> [w317 _]
                                tunnel: [w317 w318] -> w311
                                tunnel: w310 -> [_ w318]
                                frame No Error {
                                }
                                frame Error {
                                }
                              }
                            }
                          }
                        }
                      }
                    }
                  }
                }
                frame False {
                  # "no-tag mode"
                  n157 = Match Pattern(string=w506, regular expression=";") -> (offset past match=w508:i32)  [unwired: 1 in, 3 out]
                  n158 = Greater Or Equal To 0?(x=w508) -> (x >= 0?=w505:bool)
                  n159 = case shown="False" w505 {
                    tunnel: w503 -> [w513 w530]
                    tunnel: w504 -> [w512 w521]
                    tunnel: [w516 w525] -> w510
                    tunnel: [w515 w526] -> w509
                    tunnel: w506 -> [w514 w524]
                    tunnel: w502 -> [w511 w520]
                    frame False {
                      w517 = 0 ("index")
                      # "#github 23\n如果没有发现Label:Value Pair\n将String转换为第一个基础类型"
                      # "Only 1 value is found"
                      n160 = Index Array(array=w513, index=w517) -> (element=w519:variant)
                      n161 = call "Convert API String Arguments to Data(variant).vi"("Type"=w519, "error in (no error)"=w512, "Strict Label Check?(T)"=w511, "String"=w514) -> ("error"=w516:errorcluster, "Data"=w518:variant)  [unwired: 6 in]
                      n162 = Replace Array Subset(array=w513, new element=w518, index=w517) -> (w515:variant[])
                    }
                    frame True {
                      # "Multiple values are found"
                      n163 = call "Cluster API String to 1D Array(Splite Nested Cluster).vi"("error in (no error)"=w521, "trimmed string in"=w524) -> ("error out"=w522:errorcluster, "Array of Strings"=w523:string[])  [unwired: 8 in]
                      n164 = Array Size(array=w523) -> (size(s)=w529:i32)
                      n165 = Array Size(array=w530) -> (size(s)=w528:i32)
                      n166 = Max & Min(x=w529, y=w528) -> (min(x,y)=w527:i32)  [unwired: 1 out]
                      n167 = for {
                        N: w527 -> [_]
                        shift-right: [w537] -> _
                        shift-left: w523 -> [w538]
                        shift-right: [w534] -> w526
                        shift-left: w530 -> [w536]
                        shift-right: [w533] -> w525
                        shift-left: w522 -> [w532]
                        tunnel: w520 -> [w531]
                        i -> [w535]
                        n168 = in-place {
                          in-place-border: [w541] -> w533
                          in-place-border: w532 -> [w540]
                          in-place-border: w531 -> [w539]
                          n169 = in-place-array #1(w538, w535) -> (w544:string)
                          n170 = in-place-array #2(w536, w535) -> (w543:variant)
                          n171 = call "Convert API String Arguments to Data(variant).vi"("Type"=w543, "error in (no error)"=w540, "Strict Label Check?(T)"=w539, "String"=w544) -> ("error"=w541:errorcluster, "Data"=w542:variant)  [unwired: 6 in]
                          n172 = in-place-array #1(w544) -> (w537:string[])  [unwired: 1 out]
                          n173 = in-place-array #2(w542) -> (w534:variant[])  [unwired: 1 out]
                        }
                      }
                    }
                  }
                }
              }
              n174 = call "SingleElementsArray To Data_csm.vi"("Pototype"=w259, "error in (no error)"=w268, "DataElementArray"=w270) -> ("error out"=w269:errorcluster, "Cluster"=w267:variant)  [unwired: 7 in]
            }
          }
        }
        frame "Timestamp" {
          n175 = case shown="Default" w570 {
            selector: w570 -> [_ w579]
            tunnel: w573 -> [w574 w582]
            tunnel: [w575 w581] -> w572
            tunnel: [w574 w580] -> w571
            frame "" {
              # "For Timestamp, empty string will be converted to current time."
              n176 = Get Date/Time In Seconds() -> (seconds since 1Jan1904=w575:timestamp)
            }
            frame Default {
              n177 = Match Pattern(string=w579, regular expression="^[0-9a-fA-F]$") -> (offset past match=w577:i32)  [unwired: 1 in, 3 out]
              n178 = Greater Or Equal To 0?(x=w577) -> (x >= 0?=w576:bool)
              n179 = case shown="False" w576 {
                tunnel: w582 -> [w588 w608]
                tunnel: [w589 w607] -> w581
                tunnel: [w587 w606] -> w580
                tunnel: w579 -> [w592 w604]
                frame False {
                  n180 = Match Pattern(string=w592, regular expression="(") -> (before substring=w586:string, after substring=w585:string)  [unwired: 1 in, 2 out]
                  n181 = Match Pattern(string=w585, regular expression=")") -> (before substring=w584:string)  [unwired: 1 in, 3 out]
                  n182 = call <userlib>:"Trim Single-line Text.vi"("single-line text"=w584) -> ("trimed text"=w583:string)  [unwired: 2 in]
                  n183 = case shown="\"\", \"UTC\"" w583 {
                    tunnel: w586 -> [w598 w603]
                    tunnel: w584 -> [w599 _]
                    tunnel: [w595 w602] -> w589
                    tunnel: w588 -> [w594 w600]
                    tunnel: [w593 w601] -> w587
                    frame Default {
                      w596 = timestamp(0 s since 1904-01-01) ("Time Stamp")
                      n184 = Scan From String(format string=w599, input string=w598, error in=w594, default 1=w596) -> (error out=w593:errorcluster, output 1=w597:timestamp)  [unwired: 1 in, 2 out]
                      n185 = Select(t=w596, s=w593, f=w597) -> (s? t:f=w595:timestamp)
                    }
                    frame "", "UTC" {
                      n186 = call "Text to Timestamp(RFC3339).vi"("error in (no error)"=w600, "Text Timestamp"=w603) -> ("error out"=w601:errorcluster, "Time Stamp"=w602:timestamp)  [unwired: 6 in, 2 out]
                    }
                  }
                }
                frame True {
                  n187 = call <userlib>:"CSM - Convert HexStr to Data.vi"("HEX String"=w604) -> ("Variant"=w607:variant, "error out"=w605:errorcluster)  [unwired: 7 in]
                  n188 = Merge Errors(w608, w605) -> (w606:errorcluster)
                }
              }
            }
          }
        }
        frame Default {
          n189 = case shown="Default" w612 {
            selector: w612 -> [w617 _]
            tunnel: w613 -> [w618 w620]
            tunnel: [w616 w619] -> w611
            tunnel: [w615 w620] -> w610
            tunnel: w609 -> [_ w619]
            frame Default {
              n190 = call <userlib>:"CSM - Convert HexStr to Data.vi"("HEX String"=w617) -> ("Variant"=w616:variant, "error out"=w614:errorcluster)  [unwired: 7 in]
              n191 = Merge Errors(w618, w614) -> (w615:errorcluster)
            }
            frame "" {
            }
          }
        }
      }
    }
    frame Error {
    }
  }
  "Data" <- w5
  "error" <- w6
